vi "Clear Compiled Object Cache.vi"(8 "error in":errorcluster, 11 "Project Manager in":refnum<class "Project Manager.lvclass">) -> (0 "error out":errorcluster, 3 "Project Manager out":refnum<class "Project Manager.lvclass">)   [LabVIEW 2026, in "Project Manager.lvclass"]
doc: "Clear compiled object cache (as preparation for build, that is the reason why this method resides in this interface)."
uses:
  Project Manager.lvclass
  Project Manager.lvclass/Project Manager.ctl
  Interfaces/ILogger/ILogger Messages/Log Msg/Log Msg.lvclass/Log Msg.ctl
  <vilib>/ActorFramework/Message Enqueuer/Message Enqueuer.lvclass/Message Enqueuer.ctl
  <vilib>/ActorFramework/Message Enqueuer/Enqueue.vi
  Interfaces/ILogger/ILogger Messages/Log Msg/Log Msg.lvclass
  <vilib>/ActorFramework/Message Priority Queue/Priority Enqueue.vi
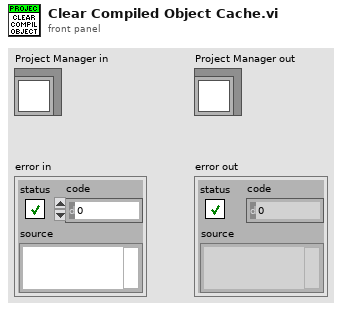
[diagram p1: front panel]
types:
  T1 = typedef "Log Entry--cluster.ctl" = cluster{"Time":timestamp, "Message":string}
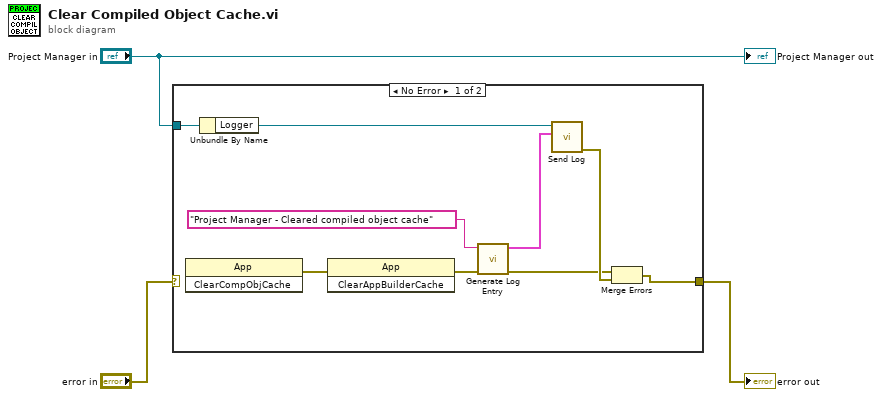
[diagram p0: block diagram]
diagram:
  n1 = case shown="No Error" "error in" {
    selector: "error in" -> [_ w13]
    tunnel: "Project Manager in" -> [w9 _]
    tunnel: [w10 w13] -> w2
    frame No Error {
      n2 = invoke class="App" method="ClearCompObjCache"() -> (error out=w5:errorcluster)  [unwired: 3 in, 2 out]
      n3 = Unbundle By Name(w9) -> ("Logger"=w7:refnum<class "Message Enqueuer.lvclass">)
      n4 = invoke class="App" method="ClearAppBuilderCache"(error in=w5) -> (error out=w4:errorcluster)  [unwired: 2 in, 2 out]
      n5 = call "Generate Log Entry.vi"("error in"=w4, "Message"="Project Manager - Cleared compiled object cache") -> ("error out"=w11:errorcluster, "Log Entry"=w6:T1)  [unwired: 8 in]
      n6 = call "Send Log.vi"("Log Entry"=w6, "Message Enqueuer"=w7) -> ("error out"=w12:errorcluster)  [unwired: 8 in, 1 out]
      n7 = Merge Errors(w11, w12) -> (w10:errorcluster)
    }
    frame Error {
      # "Pass error without further actions."
    }
  }
  "error out" <- w2
  "Project Manager out" <- "Project Manager in"
